vi "DAC Run.vi"(8 "error in":errorcluster, 11 "DAC Vacum Pressure in":refnum<class "DAC Vacum Pressure.lvclass">) -> (0 "error out":errorcluster, 3 "DAC Vacum Pressure out":refnum<class "DAC Vacum Pressure.lvclass">)   [LabVIEW 2019, in "DAC.lvlib" / "DAC Vacum Pressure.lvclass"]
uses:
  DAC Vacum Pressure.lvclass
  C:/Users/krio/Documents/LV_Projects/test-stand/App/DAC/DAC.lvclass
  DAC.lvclass/DAC.ctl
  Results/HTS Results/HTS Results.lvclass
  Results/Results Method.ctl
  DAC Vacum Pressure.lvclass/DAC Vacum Pressure.ctl
  Results/HTS Results/HTS Results.lvclass/HTS Results.ctl
  <vilib>/DAQmx/read.llb/DAQmx Read (Analog DBL 1Chan 1Samp).vi
  <vilib>/DAQmx/miscellaneous.llb/DAQmx Fill In Error Info.vi
  DAC.lvclass
  Results/Results.lvlib
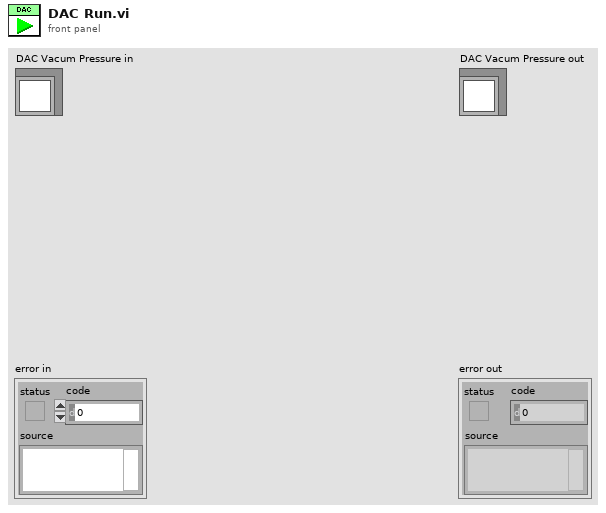
[diagram p1: front panel]
types:
  T1 = typedef "Results.lvlib/Results Method.ctl" = enum16{"Get", "Set"}
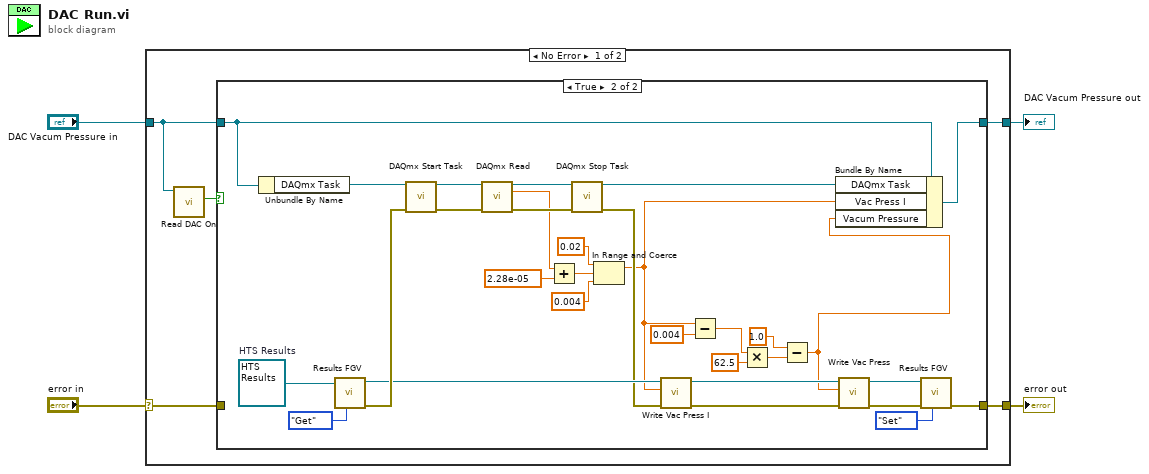
[diagram p0: block diagram]
diagram:
  n1 = case shown="No Error" "error in" {
    selector: "error in" -> [w7 w44]
    tunnel: [w6 w44] -> w2
    tunnel: [w8 w43] -> w1
    tunnel: "DAC Vacum Pressure in" -> [w5 w43]
    frame No Error {
      n2 = call "Read DAC On.vi"("DAC in"=w5) -> ("DAC On"=w9:bool)  [unwired: 8 in, 2 out]
      n3 = case shown="True" w9 {
        tunnel: w5 -> [w11 w38]
        tunnel: [w11 w31] -> w8
        tunnel: w7 -> [w10 _]
        tunnel: [w10 w30] -> w6
        frame False {
        }
        frame True {
          w37 = refnum<class "HTS Results.lvclass"> refnum  # HTS Results
          n4 = Unbundle By Name(w38) -> ("DAQmx Task"=w42:refnum<k21>)
          n5 = call-dynamic "Results FGV.vi"("Method"=Results_Method."Get", "HTS Results in"=w37) -> ("error out"=w34:errorcluster, "HTS Results out"=w24:refnum<class "HTS Results.lvclass">)  [unwired: 8 in]
          n6 = call <vilib>:"DAQmx Start Task.vi"("task/channels in"=w42, "error in"=w34) -> ("task out"=w41:refnum<k21>, "error out"=w40:errorcluster)  [unwired: 12 in]
          n7 = call-poly <vilib>:"DAQmx Read.vi"("task/channels in"=w41, "error in"=w40) -> ("task out"=w32:refnum<k21>, "data"=w20:dbl, "error out"=w39:errorcluster)  [unwired: 11 in]
          n8 = Add(x=w20, y=2.28e-05) -> (x+y=w18:dbl)
          n9 = call <vilib>:"DAQmx Stop Task.vi"("task/channels in"=w32, "error in"=w39) -> ("task out"=w33:refnum<k21>, "error out"=w21:errorcluster)  [unwired: 12 in]
          n10 = In Range and Coerce(upper limit=0.02, x=w18, lower limit=0.004) -> (coerced(x)=w17:dbl)  [unwired: 1 out]
          n11 = call "Write Vac Press I.vi"("error in (no error)"=w21, "Vac Press I"=w17, "HTS Results in"=w24) -> ("error out"=w22:errorcluster, "HTS Results out"=w23:refnum<class "HTS Results.lvclass">)  [unwired: 7 in]
          n12 = Subtract(x=w17, y=0.004) -> (x-y=w28:dbl)
          n13 = Multiply(x=w28, y=62.5) -> (x*y=w14:dbl)
          n14 = Subtract(x=1.0, y=w14) -> (x-y=w12:dbl)
          n15 = Bundle By Name(cluster=w38, "DAQmx Task"=w33, "Vac Press I"=w17, "Vacum Pressure"=w12) -> (w31:refnum<class "DAC Vacum Pressure.lvclass">)
          n16 = call "Write Vac Press.vi"("error in (no error)"=w22, "Vac Press"=w12, "HTS Results in"=w23) -> ("error out"=w25:errorcluster, "HTS Results out"=w26:refnum<class "HTS Results.lvclass">)  [unwired: 7 in]
          n17 = call-dynamic "Results FGV.vi"("Method"=Results_Method."Set", "error in"=w25, "HTS Results in"=w26) -> ("error out"=w30:errorcluster)  [unwired: 7 in, 1 out]
        }
      }
    }
    frame Error {
    }
  }
  "error out" <- w2
  "DAC Vacum Pressure out" <- w1
